vi "Position Error FeedForward.vi"(6 "Position Error":dbl=-0.014062500000000089) -> (7 "?":dbl=-0.0)   [LabVIEW 2027]
panel:
  in  "Power Addition (In Volts)":dbl=-0.4 format="%#_13g"
  # "Feed Forward Addition"
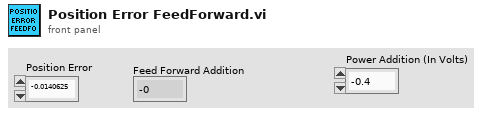
[diagram p1: front panel]
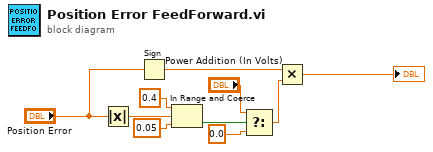
[diagram p0: block diagram]
diagram:
  n1 = Absolute Value(x="Position Error") -> (abs(x)=w9:dbl)
  n2 = Sign(1:"Position Error") -> (0:w8:dbl)
  n3 = In Range and Coerce(upper limit=0.4, x=w9, lower limit=0.05) -> (In Range?=w5:bool)  [unwired: 1 out]
  n4 = Select(t="Power Addition (In Volts)", s=w5, f=0.0) -> (s? t:f=w10:dbl)
  n5 = Multiply(x=w8, y=w10) -> (x*y=→"?":dbl)
